vi "HandShaking.vi"(6 "Elapsed Time":u32, 8 "error in":errorcluster, 9 "Sequence Context":refnum<k7>, 10 "Stop":refnum<user-event>, 11 "PostUUT in":refnum<class "PostUUT.lvclass">=refnum) -> (0 "error out":errorcluster, 3 "PostUUT out":refnum<class "PostUUT.lvclass">)   [LabVIEW 2025, in "PostUUT.lvclass"]
uses:
  PostUUT.lvclass
  C:/Working copy/TS Manager/Plugin/Tests/Submodule EOL/TS Execution Interface/OPC UA/Abstract.lvclass
  e5edfce7-0da4-434f-8ef9-908b5fb189e7.vi
  OPC UA/Read Rx from PLC.vi
  OPC UA/Read Tx to PLC.vi
  <vilib>/addons/TestStand/_TSUtility.llb/TestStand - Get Property Value (String).vi
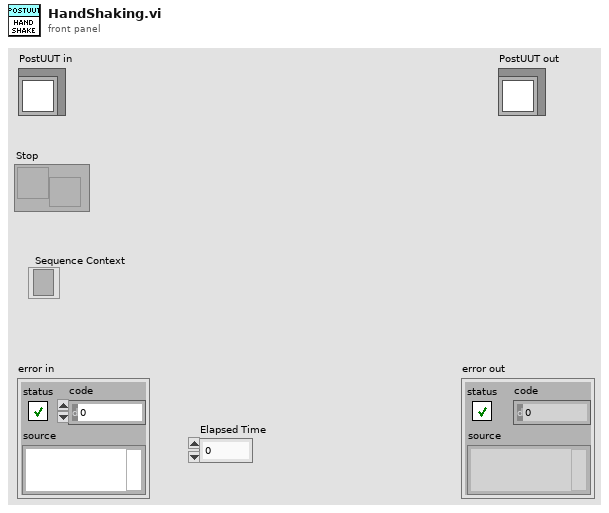
[diagram p1: front panel]
types:
  T1 = typedef "OPC UA.lvlib/OPC UA.lvclass/Tester Rx Dataset.ctl" = cluster{"Start":bool, "NestStatus":bool, "PalletID":u32, "BarcodeData":string, "StepEcho":u32, "Cylinder_1":bool, "Cylinder_2":bool, "Cylinder_3":bool, "Cylinder_4":bool, "Cylinder_5":bool, "ResultsAck":bool, "Reset":bool, "Stop":bool, "FaultCode":u32}
  T2 = typedef "OPC UA.lvlib/OPC UA.lvclass/Tester Tx Dataset.ctl" = cluster{"Fault":bool, "StepNo":u32, "Ready":bool, "HighVoltage":bool, "TestRunning":bool, "ResultsReady":bool, "Results":u32, "ElapsedTime":u32, "Online":bool, "TimeCompleted":i32[], "Timeout":bool, "Heartbeat":bool}
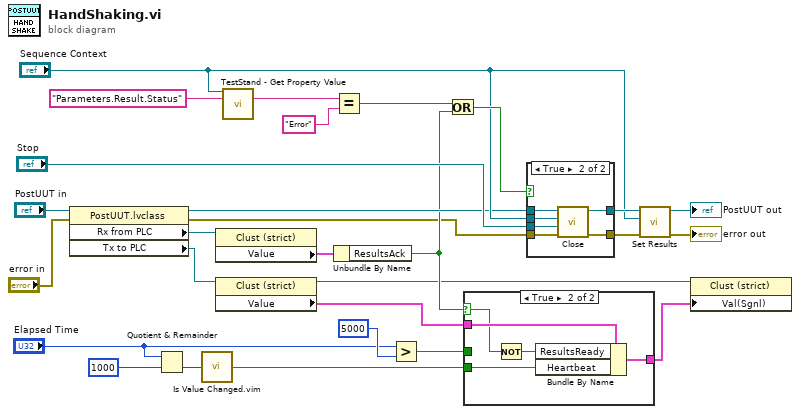
[diagram p0: block diagram]
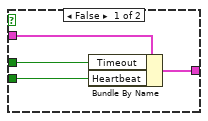
[diagram p2: hidden frame]
diagram:
  n1 = property class="PostUUT.lvclass"(reference="PostUUT in", error in="error in") -> (reference out=w8:refnum<class "PostUUT.lvclass">, error out=w1:errorcluster, "Rx from PLC"=w3:refnum<vi>, "Tx to PLC"=w4:refnum<vi>)
  n2 = Quotient & Remainder(x="Elapsed Time", y=u32 1000) -> (floor(x/y)=w23:u32)  [unwired: 1 out]
  n3 = call "Is Value Changed.vim"("value"=w23) -> ("changed or first call?"=w21:bool)
  n4 = property class="Clust (strict)"(reference=w3) -> ("Value"=w27:T1)  [unwired: 1 in, 2 out]
  n5 = property class="Clust (strict)"(reference=w4) -> (reference out=w5:refnum<vi>, "Value"=w28:T2)  [unwired: 1 in, 1 out]
  n6 = call-poly <vilib>:"TestStand - Get Property Value.vi"("Sequence Context In"="Sequence Context", "Lookup String"="Parameters.Result.Status") -> ("Value"=w17:string)  [unwired: 11 in, 2 out]
  n7 = Equal?(x=w17, y="Error" ("Lookup String")) -> (x = y?=w6:bool)
  n8 = Unbundle By Name(w27) -> ("ResultsAck"=w7:bool)
  n9 = Greater?(x="Elapsed Time", y=u32 5000) -> (0:w25:bool)
  n10 = Or(x=w6, y=w7) -> (x .or. y?=w13:bool)
  n11 = case shown="True" w7 {
    selector: w7 -> [_ w36]
    tunnel: w28 -> [w32 w37]
    tunnel: [w31 w34] -> w10
    tunnel: w25 -> [w30 _]
    tunnel: w21 -> [w29 w35]
    frame False {
      n12 = Bundle By Name(cluster=w32, "Timeout"=w30, "Heartbeat"=w29) -> (w31:T2)
    }
    frame True {
      n13 = Not(x=w36) -> (.not. x?=w33:bool)
      n14 = Bundle By Name(cluster=w37, "ResultsReady"=w33, "Heartbeat"=w35) -> (w34:T2)
    }
  }
  n15 = case shown="True" w13 {
    tunnel: "Stop" -> [_ w44]
    tunnel: [w38 w45] -> w11
    tunnel: w8 -> [w39 w43]
    tunnel: [w39 w42] -> w15
    tunnel: "Sequence Context" -> [_ w41]
    tunnel: w1 -> [w38 w40]
    frame False {
    }
    frame True {
      n16 = call-dynamic "Close.vi"("error in (no error)"=w40, "Stop Event"=w44, "Sequence Context"=w41, "Abstract"=w43) -> ("error out"=w45:errorcluster, "Abstract out"=w42:refnum<class "PostUUT.lvclass">)  [unwired: 6 in]
    }
  }
  n17 = call "Set Results.vi"("error in"=w11, "Sequence Context"="Sequence Context", "PostUUT"=w15) -> ("error out"=→"error out":errorcluster, "PostUUT out"=→"PostUUT out":refnum<class "PostUUT.lvclass">)  [unwired: 7 in]
  n18 = property class="Clust (strict)"(reference=w5, "Val(Sgnl)"=w10) -> ()  [unwired: 1 in, 2 out]
